vi "WLAN_SuperposedFrameBuild_V2.vi"(4 "Modulation parameter LP":T1, 6 "OFDMON":bool, 7 "Alpha":dbl min=0.0 max=1.0 step=0.05 format="%#_13g", 8 "error in (no error)":errorcluster, 9 "data in 2":i8[](array[numeric]) caption="input bit stream", 10 "Modulation parameter HP":T1, 11 "data in":i8[](array[numeric]) caption="input bit stream") -> (0 "error out":errorcluster, 3 "output array":cdb[](array[numeric]))   [LabVIEW 2022 SP3]
panel:
  out "size(s) 6":i32
  out "size(s) 5":i32
  out "size(s) 4":i32
  out "size(s) 3":i32
  out "size(s) 2":i32
  out "size(s)":i32
  out "Encoded bits target HP":dbl
  out "Encoded bits target LP":dbl
  in  "N sym common":dbl=1484.0 min=0.0 max=1.0 step=0.05
  in  "data in 3":i8[](array[numeric]) caption="input bit stream"
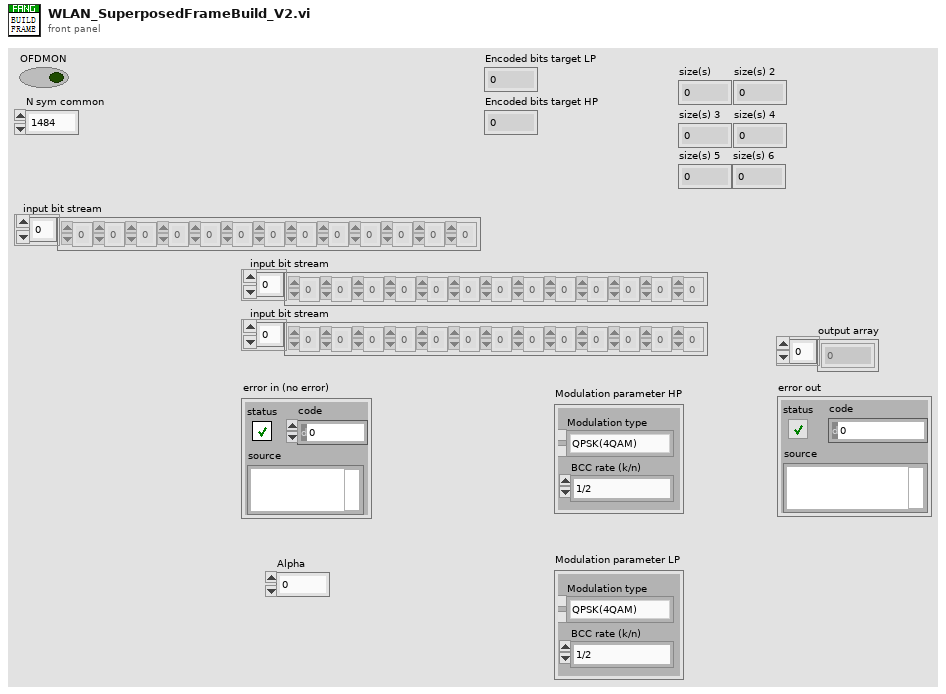
[diagram p1: front panel]
types:
  T1 = cluster{"Modulation type":enum16{"QPSK(4QAM)", "64QAM", "16QAM", "BPSK"}, "BCC rate (k/n)":enum16{"1/2", "2/3", "3/4"}}
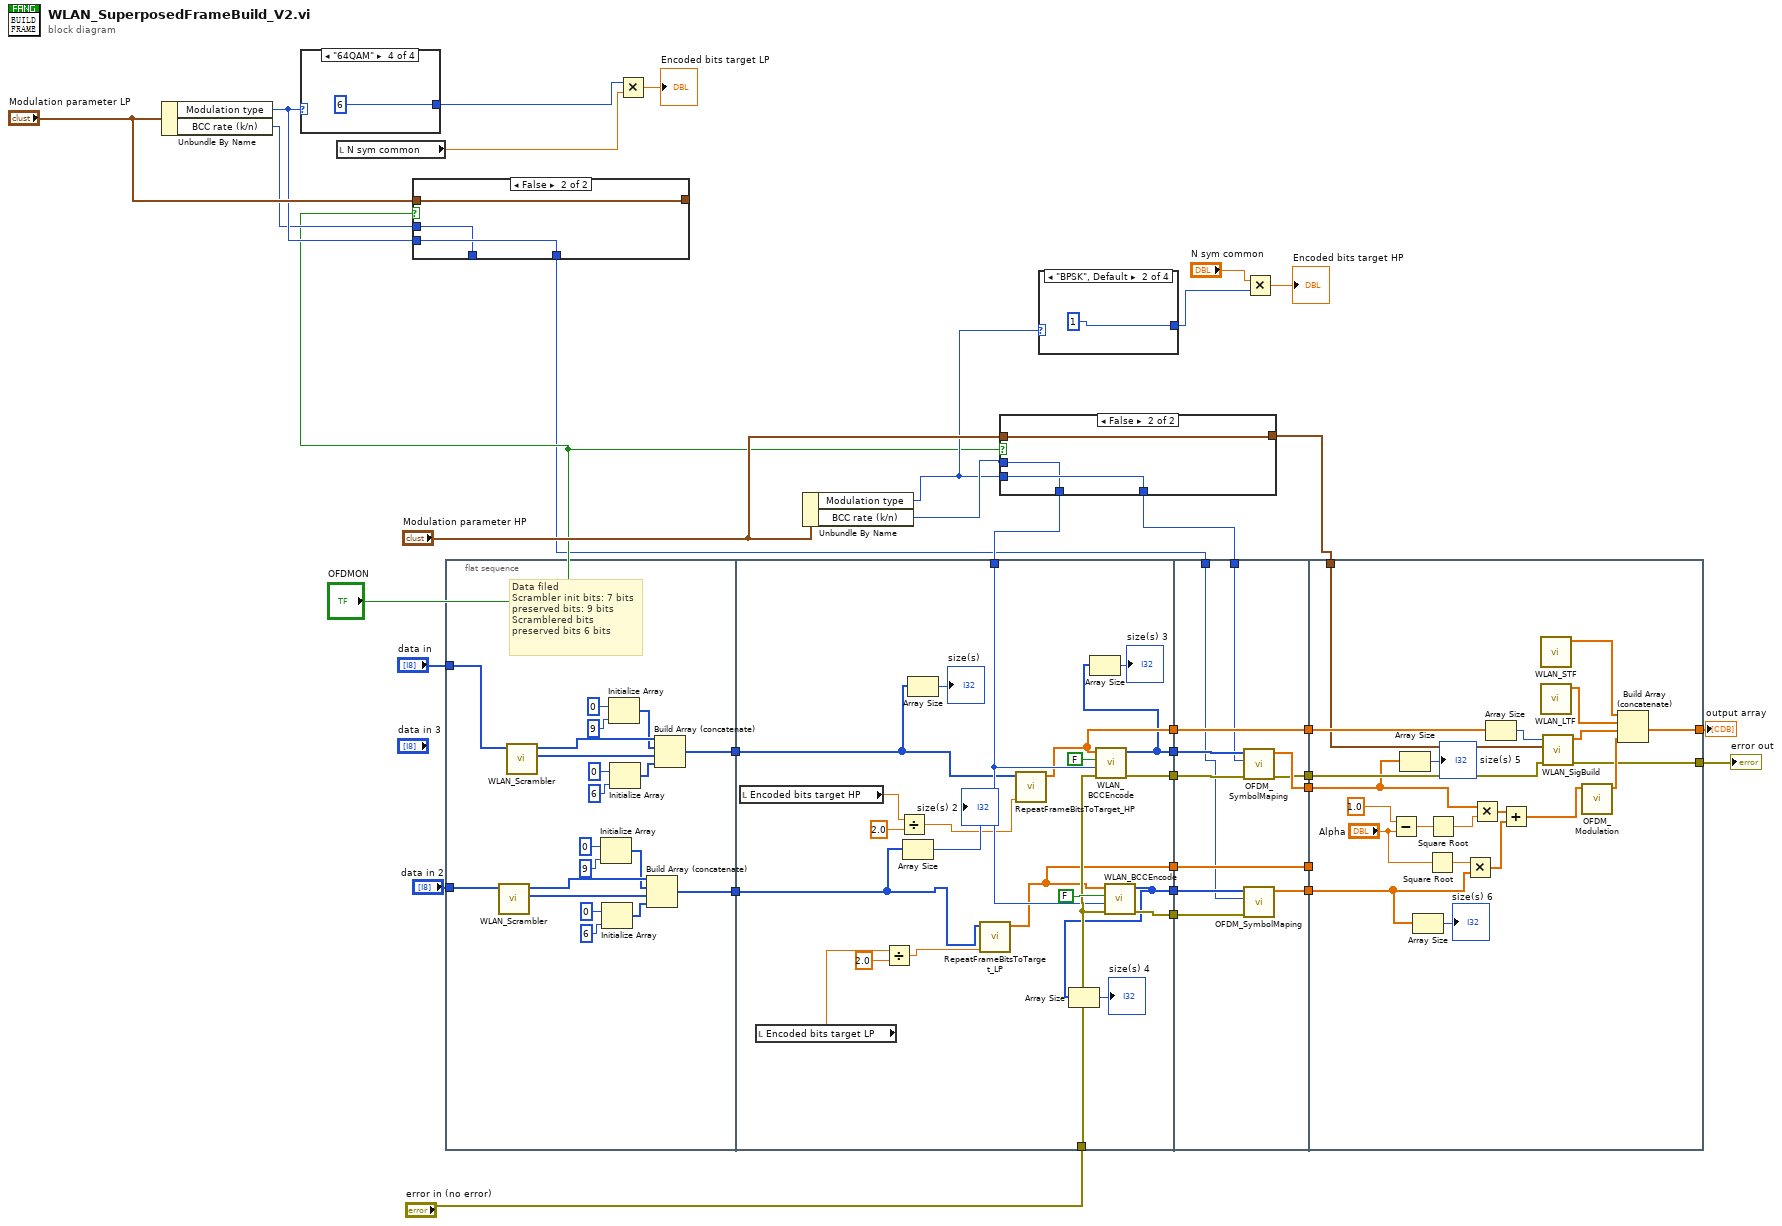
[diagram p0: block diagram]
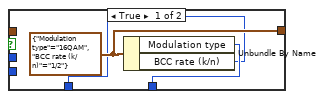
[diagram p2: hidden frame]
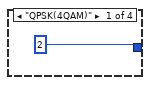
[diagram p3: hidden frame]
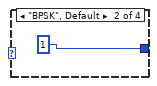
[diagram p4: hidden frame]
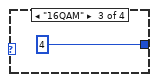
[diagram p5: hidden frame]
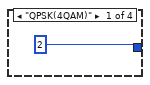
[diagram p6: hidden frame]
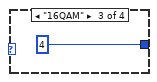
[diagram p7: hidden frame]
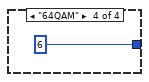
[diagram p8: hidden frame]
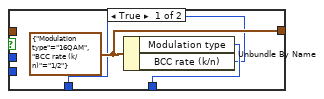
[diagram p9: hidden frame]
diagram:
  n1 = Unbundle By Name("Modulation parameter LP") -> ("Modulation type"=w4:enum16{"QPSK(4QAM)", "64QAM", "16QAM", "BPSK"}, "BCC rate (k/n)"=w3:enum16{"1/2", "2/3", "3/4"})
  n2 = case shown="\"64QAM\"" w4 {
    tunnel: [2 1 4 6] -> w9
    frame "QPSK(4QAM)" {
    }
    frame "BPSK", Default {
    }
    frame "16QAM" {
    }
    frame "64QAM" {
    }
  }
  n3 = local read "N sym common"() -> (w6:dbl)
  n4 = case shown="False" "OFDMON" {
    tunnel: w4 -> [_ w45]
    tunnel: [w42 w45] -> w1
    tunnel: [w41 w44] -> _
    tunnel: "Modulation parameter LP" -> [_ w44]
    tunnel: [w40 w43] -> _
    tunnel: w3 -> [_ w43]
    frame True {
      w41 = T1 {"Modulation type"=enum."16QAM", "BCC rate (k/n)"=enum."1/2"} ("Modulation parameter")
      n5 = Unbundle By Name(w41) -> ("Modulation type"=w42:enum16{"QPSK(4QAM)", "64QAM", "16QAM", "BPSK"}, "BCC rate (k/n)"=w40:enum16{"1/2", "2/3", "3/4"})
    }
    frame False {
    }
  }
  n6 = flat-sequence {
    tunnel: "data in" -> [w57]
    tunnel: [w56] -> w34
    tunnel: "data in 2" -> [w47]
    tunnel: [w46] -> w23
    tunnel: w34 -> [w81]
    tunnel: "error in (no error)" -> [w84]
    tunnel: [w86] -> w32
    tunnel: [w75] -> w31
    tunnel: w14 -> [w83]
    tunnel: [w80] -> w26
    tunnel: w23 -> [w73]
    tunnel: [w72] -> w22
    tunnel: [w74] -> w21
    tunnel: [w82] -> w19
    tunnel: w32 -> [w98]
    tunnel: w31 -> [w97]
    tunnel: w17 -> [w89]
    tunnel: [w96] -> w30
    tunnel: [w95] -> w29
    tunnel: w26 -> [w94]
    tunnel: [w94] -> w25
    tunnel: w22 -> [w92]
    tunnel: w21 -> [w93]
    tunnel: [w92] -> w20
    tunnel: w19 -> [w91]
    tunnel: [w90] -> w18
    tunnel: w1 -> [w88]
    tunnel: w16 -> [w118]
    tunnel: w30 -> [w102]
    tunnel: w29 -> [w113]
    tunnel: [w112] -> w28
    tunnel: [w111] -> w27
    tunnel: w25 -> [w120]
    tunnel: w20 -> [_]
    tunnel: w18 -> [w100]
    frame #0 {
      # "Data filed\nScrambler init bits: 7 bits\npreserved bits: 9 bits\nScramblered bits\npreserved bits 6 bits"
      n7 = call "WLAN_Scrambler.vi"("input bit stream"=w47) -> ("scrambled bits"=w51:i8[], "scrambler initial bit"=w55:i8[])  [unwired: 9 in]
      n8 = call "WLAN_Scrambler.vi"("input bit stream"=w57) -> ("scrambled bits"=w61:i8[], "scrambler initial bit"=w65:i8[])  [unwired: 9 in]
      n9 = Initialize Array(i8 0 ("element"), 9 ("dimension size")) -> (w54:i8[])
      n10 = Initialize Array(i8 0 ("element"), 6 ("dimension size")) -> (w48:i8[])
      n11 = Initialize Array(i8 0 ("element"), 9 ("dimension size")) -> (w64:i8[])
      n12 = Initialize Array(i8 0 ("element"), 6 ("dimension size")) -> (w58:i8[])
      n13 = Build Array (concatenate)(w55, w54, w51, w48) -> (w46:i8[])
      n14 = Build Array (concatenate)(w65, w64, w61, w58) -> (w56:i8[])
    }
    frame #1 {
      n15 = local read "Encoded bits target HP"() -> (w67:dbl)
      n16 = local read "Encoded bits target LP"() -> (w70:dbl)
      n17 = Divide(x=w70, y=2.0) -> (x/y=w71:dbl)
      n18 = Divide(x=w67, y=2.0) -> (x/y=w66:dbl)
      n19 = Array Size(array=w73) -> (size(s)=→"size(s) 2":i32)
      n20 = Array Size(array=w81) -> (size(s)=→"size(s)":i32)
      n21 = call "RepeatFrameBitsToTarget_LP.vi"("target length"=w71, "bit array in"=w73) -> ("bit array out"=w72:dbl[])  [unwired: 9 in]
      n22 = call "RepeatFrameBitsToTarget_HP.vi"("target length"=w66, "bit array in"=w81) -> ("bit array out"=w80:dbl[])  [unwired: 9 in]
      n23 = call "WLAN_BCCEncode.vi"("error in (no error)"=w84, "BCC rate (k/n)"=w83, "need add zeros?"=FALSE, "input bit stream"=w80) -> ("error out"=w86:errorcluster, "output bit stream 3"=w75:i8[])  [unwired: 6 in]
      n24 = Array Size(array=w75) -> (size(s)=→"size(s) 3":i32)
      n25 = call "WLAN_BCCEncode.vi"("error in (no error)"=w84, "BCC rate (k/n)"=w83, "need add zeros?"=FALSE, "input bit stream"=w72) -> ("error out"=w82:errorcluster, "output bit stream 3"=w74:i8[])  [unwired: 6 in]
      n26 = Array Size(array=w74) -> (size(s)=→"size(s) 4":i32)
    }
    frame #2 {
      n27 = call "OFDM_SymbolMaping.vi"("error in (no error)"=w98, "Modulation type"=w89, "input bit stream"=w97) -> ("error out"=w95:errorcluster, "symbols"=w96:cdb[])  [unwired: 7 in]
      n28 = call "OFDM_SymbolMaping.vi"("error in (no error)"=w91, "Modulation type"=w88, "input bit stream"=w93) -> ("symbols"=w90:cdb[])  [unwired: 7 in, 1 out]
    }
    frame #3 {
      n29 = Subtract(x=1.0, y="Alpha") -> (x-y=w105:dbl)
      n30 = Array Size(array=w102) -> (size(s)=→"size(s) 5":i32)
      n31 = Array Size(array=w100) -> (size(s)=→"size(s) 6":i32)
      n32 = Square Root(x="Alpha") -> (sqrt(x)=w109:dbl)
      n33 = Square Root(x=w105) -> (sqrt(x)=w107:dbl)
      n34 = Multiply(x=w109, y=w100) -> (x*y=w110:cdb[])
      n35 = Multiply(x=w102, y=w107) -> (x*y=w108:cdb[])
      n36 = Array Size(array=w120) -> (size(s)=w119:i32)
      n37 = Add(x=w108, y=w110) -> (x+y=w103:cdb[])
      n38 = call "WLAN_STF.vi"() -> ("STF"=w114:cdb[])  [unwired: 11 in]
      n39 = call "WLAN_LTF.vi"() -> ("LTF"=w115:cdb[])  [unwired: 11 in]
      n40 = call "WLAN_SigBuild.vi"("Data bit length"=w119, "Modulation parameter"=w118, "error in (no error)"=w113) -> ("symbols"=w116:cdb[], "error out"=w112:errorcluster)  [unwired: 6 in]
      n41 = call "OFDM_Modulation.vi"("Input sequence"=w103) -> ("Output sequence"=w117:cdb[])  [unwired: 10 in]
      n42 = Build Array (concatenate)(w114, w115, w116, w117) -> (w111:cdb[])
    }
  }
  n43 = Multiply(x=w9, y=w6) -> (x*y=→"Encoded bits target LP":dbl)
  n44 = Unbundle By Name("Modulation parameter HP") -> ("Modulation type"=w12:enum16{"QPSK(4QAM)", "64QAM", "16QAM", "BPSK"}, "BCC rate (k/n)"=w13:enum16{"1/2", "2/3", "3/4"})
  n45 = case shown="False" "OFDMON" {
    tunnel: w12 -> [_ w126]
    tunnel: [w123 w126] -> w17
    tunnel: [w122 w125] -> w16
    tunnel: "Modulation parameter HP" -> [_ w125]
    tunnel: [w121 w124] -> w14
    tunnel: w13 -> [_ w124]
    frame True {
      w122 = T1 {"Modulation type"=enum."16QAM", "BCC rate (k/n)"=enum."1/2"} ("Modulation parameter")
      n46 = Unbundle By Name(w122) -> ("Modulation type"=w123:enum16{"QPSK(4QAM)", "64QAM", "16QAM", "BPSK"}, "BCC rate (k/n)"=w121:enum16{"1/2", "2/3", "3/4"})
    }
    frame False {
    }
  }
  n47 = case shown="\"BPSK\", Default" w12 {
    tunnel: [2 1 4 6] -> w8
    frame "QPSK(4QAM)" {
    }
    frame "BPSK", Default {
    }
    frame "16QAM" {
    }
    frame "64QAM" {
    }
  }
  n48 = Multiply(x="N sym common", y=w8) -> (x*y=→"Encoded bits target HP":dbl)
  "output array" <- w27
  "error out" <- w28
